vi "Lab4_task4.vi"() -> ()   [LabVIEW 2022 SP3]
uses:
  <vilib>/express/express analysis/Spectral/Block/exnSpectralBlock spectral measurements PSD poly.vi
  <vilib>/express/express analysis/Spectral/Block/exnSpectralBlock spectral measurements PSD DDT.vi
  <vilib>/express/express analysis/Spectral/XNode/ExpressSpectralMeasurementsBlockNode.xnode
panel:
  out "Array":dbl[](array[numeric])
  out "Intensity Chart":dbl[][](graph)
  in  "stop":bool
  in  "number of samples":i32=100000
  out "PSD":dynamicdata(graph)
  in  "Sampling rate (Hz)":dbl
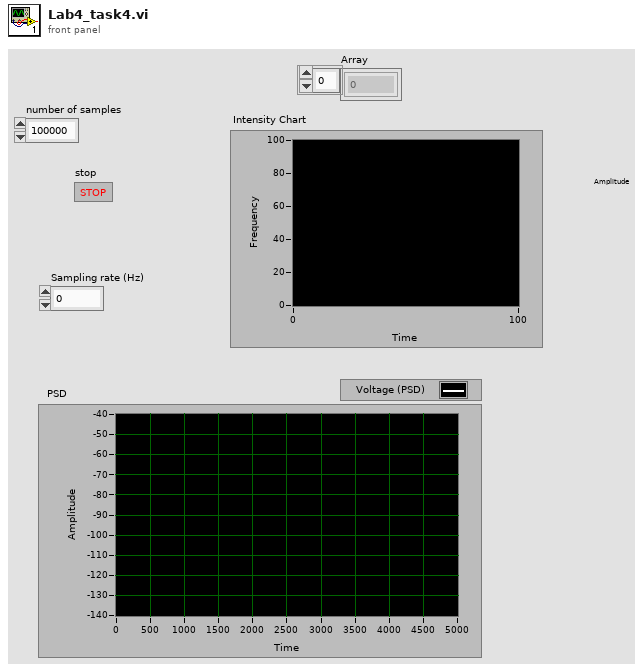
[diagram p1: front panel]
types:
  T1 = cluster{"averaging mode":u16, "weighting mode":u16, "number of averages":u32}
  T2 = cluster{"dB On (F)":bool, "unwrap phase (F)":bool, "convert to degree (F)":bool}
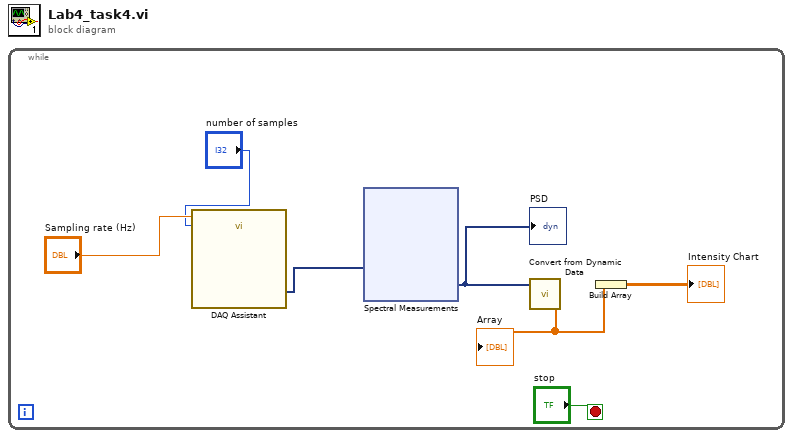
[diagram p0: block diagram]
diagram:
  n1 = while {
    stop <- "stop" stop-if-true
    n2 = call "DAQ Assistant"("rate"="Sampling rate (Hz)", "number of samples"="number of samples") -> ("data"=w5:dynamicdata)  [unwired: 15 in, 2 out]
    n3 = xnode "Spectral Measurements"("Signals"=w5) -> ("PSD"=w3:dynamicdata)  [unwired: 1 in, 1 out]
    "PSD" <- w3
    n4 = call "Convert from Dynamic Data"("Dynamic Data Type"=w3) -> ("Array"=w2:dbl[])  [unwired: 3 in]
    "Array" <- w2
    n5 = Build Array(w2) -> (→"Intensity Chart":dbl[][])
  }
